vi "Write baud rate.vi"(8 "error in (no error)":errorcluster, 10 "baud rate":u32=9600, 11 "Modbus_RTU in":refnum<class "Modbus_RTU.lvclass">) -> (0 "error out":errorcluster, 3 "Modbus_RTU out":refnum<class "Modbus_RTU.lvclass">)   [LabVIEW 2021, in "Modbus_RTU.lvclass"]
uses:
  Modbus_RTU.lvclass
  Modbus_RTU.lvclass/Modbus_RTU.ctl
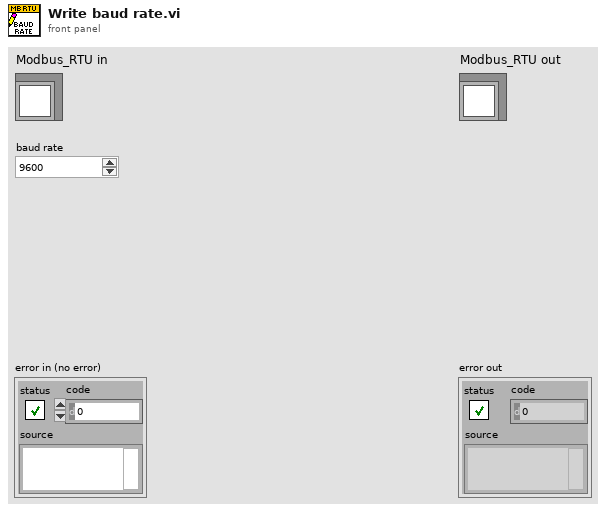
[diagram p1: front panel]
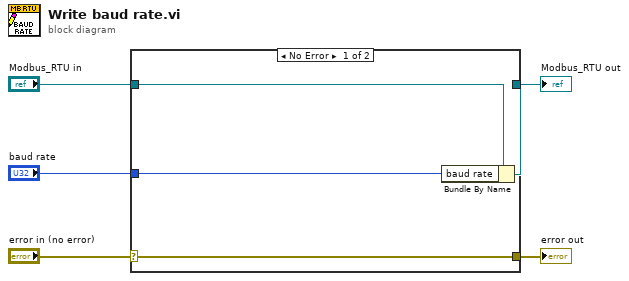
[diagram p0: block diagram]
diagram:
  n1 = case shown="No Error" "error in (no error)" {
    selector: "error in (no error)" -> [w9 w10]
    tunnel: [w9 w10] -> w4
    tunnel: [w7 w11] -> w2
    tunnel: "Modbus_RTU in" -> [w8 w11]
    tunnel: "baud rate" -> [w6 _]
    frame No Error {
      n2 = Bundle By Name(cluster=w8, "baud rate"=w6) -> (w7:refnum<class "Modbus_RTU.lvclass">)
    }
    frame Error {
    }
  }
  "error out" <- w4
  "Modbus_RTU out" <- w2
